vi "CP Selection for Plot and Graph_MS.vi"(7 "Sample cluster":T2, 8 "CP Profile Table":string[][](table), 9 "CP A Tag":string[](array[string]), 10 "Signal Tag AZ":string[](array[string]), 11 "Long Signal Profile Table A":string[][](table) caption="Long Singla Profile Table") -> (0 "CP A Tag AZ":string[](array[string]), 1 "Abs Plot Graph":dbl[][](graph), 2 "Plot Graph":dbl[][](graph), 3 "LCP Table":string[][](table), 5 "LAP":T1)   [LabVIEW 2018]
panel:
  out "LAP_Tag":string[](array[string])
  out "LAP Table":string[][](table) caption="LCP Table"
  out "M_Base Number":i32[](array[numeric])
  out "Direction":string[](array[string])
  out "Cutted Sequence":string
  out "Sample Sequence":string
  out "M_Seq EN":i32
  out "M_Seq SN":i32
  out "LS#":string[][](array[string])
  out "CP Profile Table for Bseq":string[][](table)
  out "CP Profile Table for All Seql":string[][](table)
  out "CP Profile Table for RSeq":string[][](table)
  out "読み取り開始番号":i32
  out "読み取り終了番号":i32
  out "Base Number":i32[](array[numeric])
  out "Seq EN":i32
  out "Seq SN":i32
  out "サイズ":i32
  out "Signal Profile Table":string[][](table) caption="Singla Profile Table"
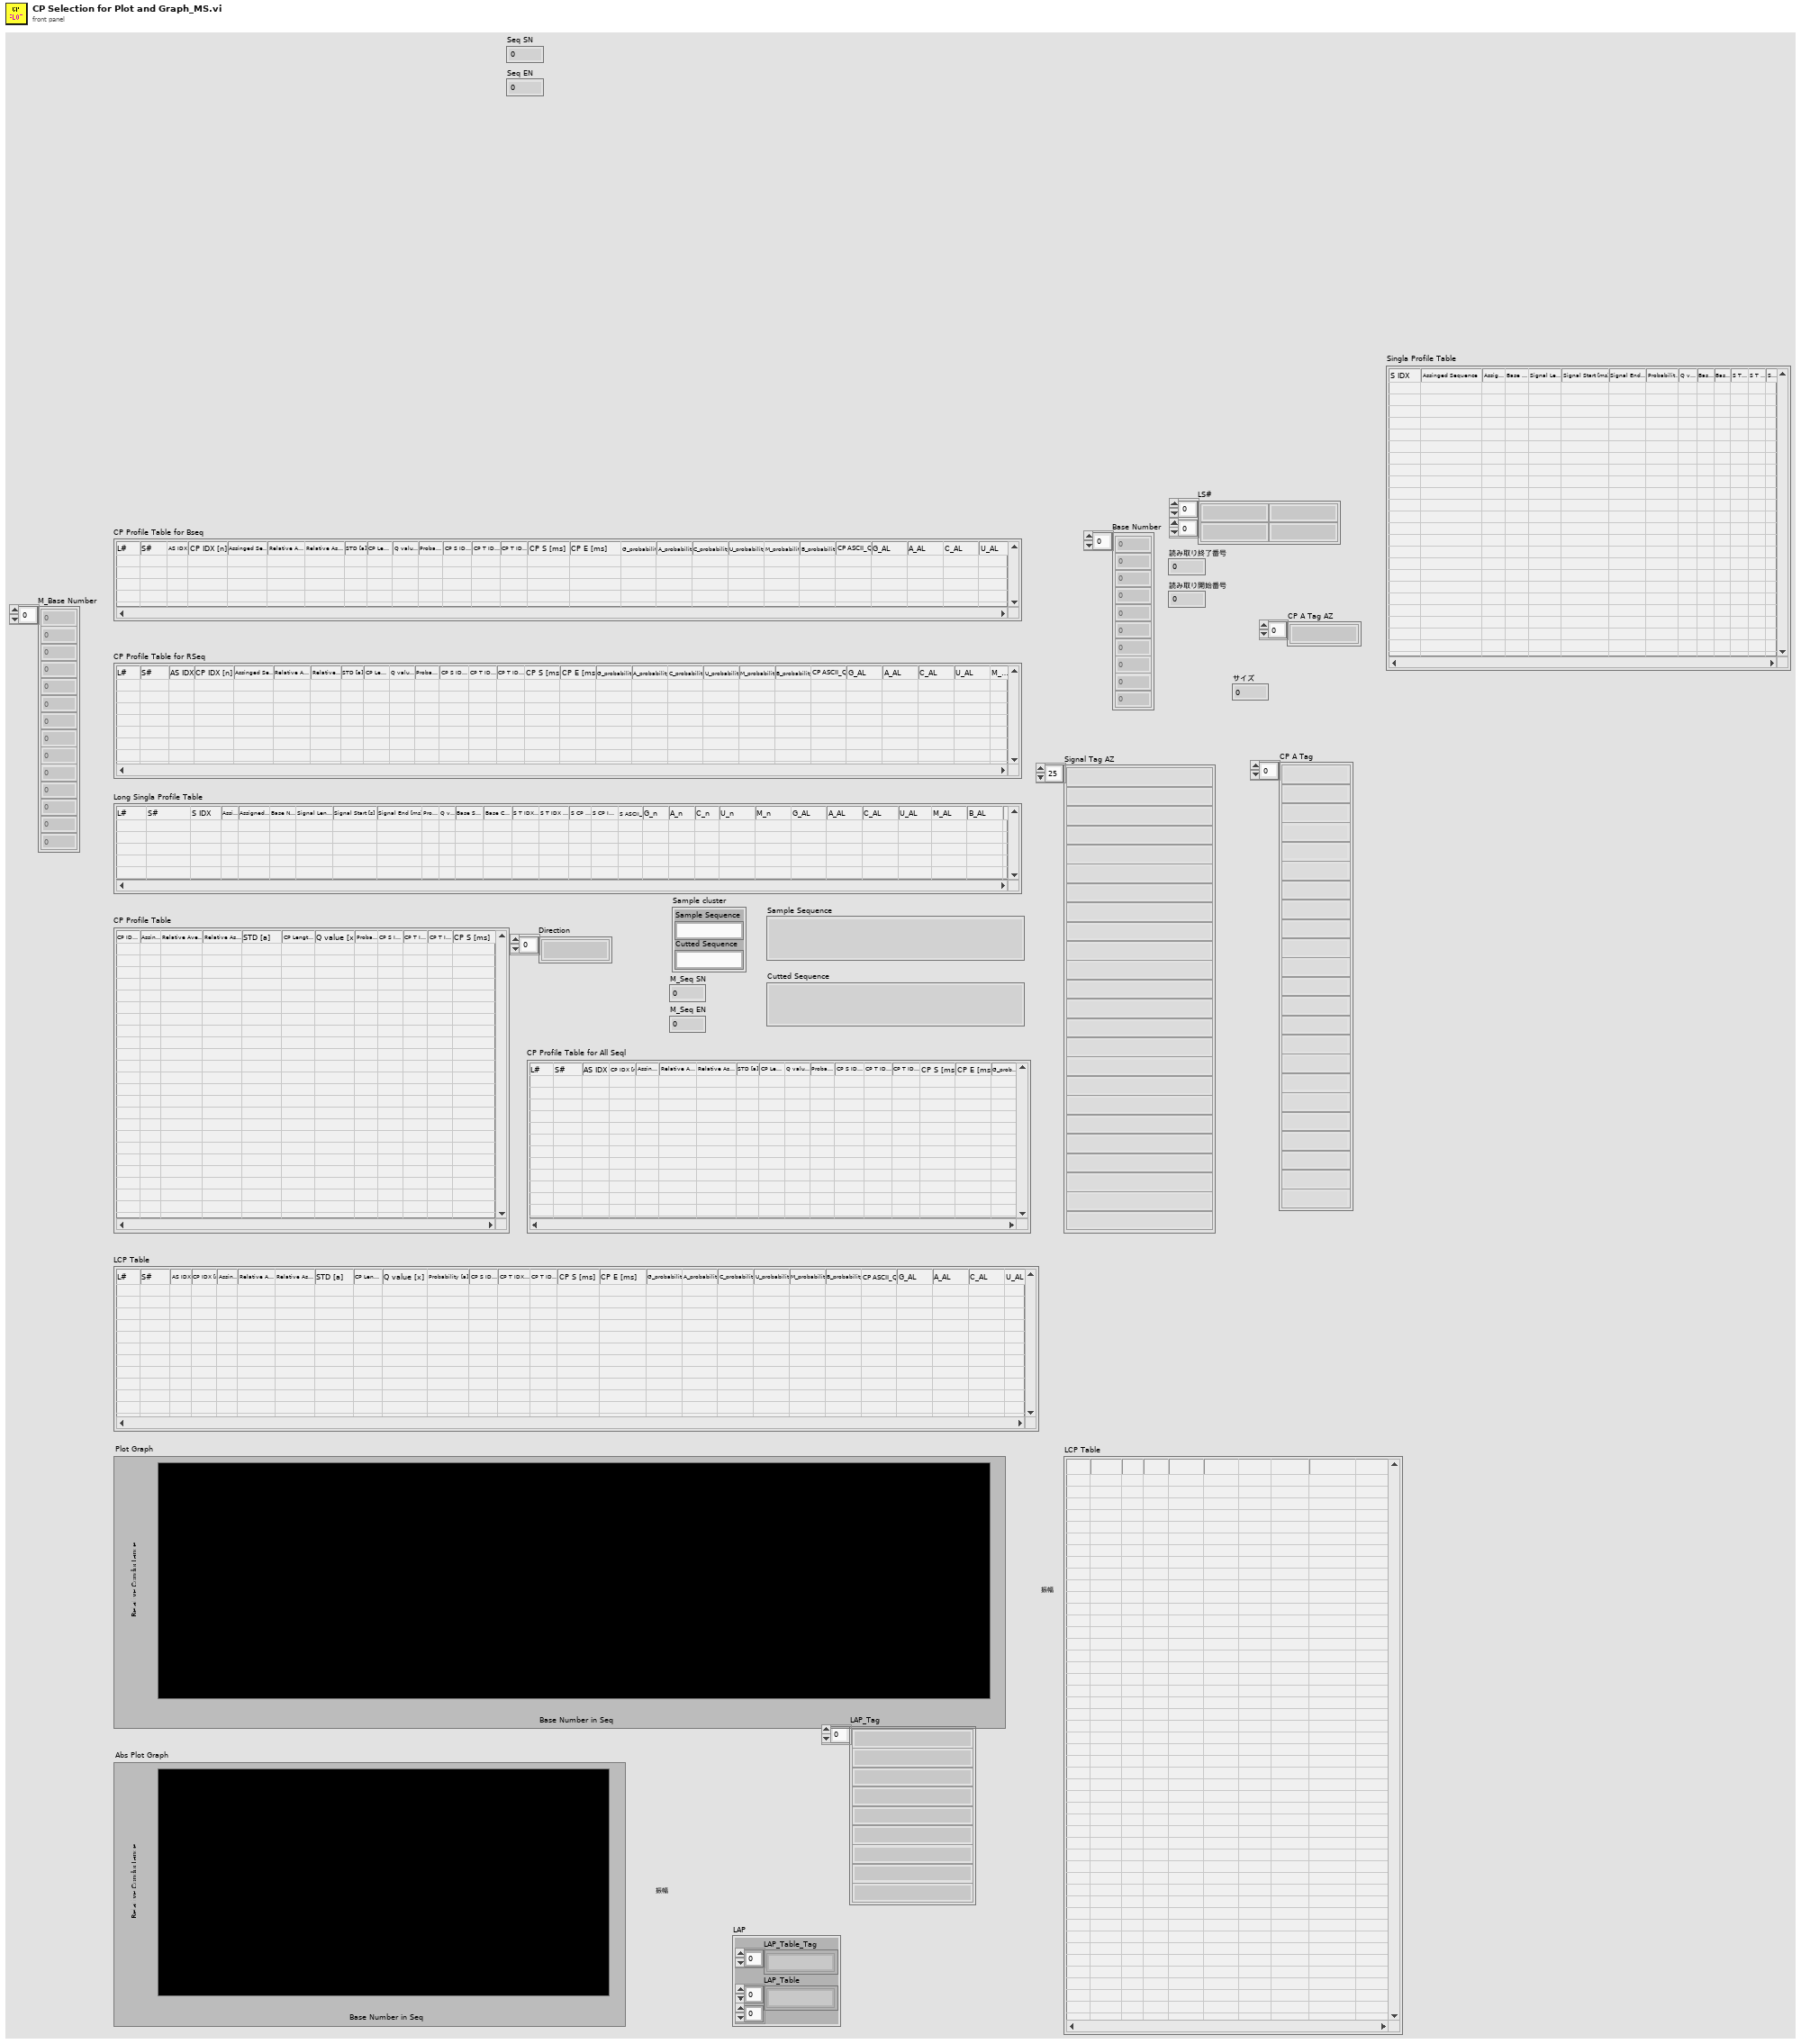
[diagram p1: front panel]
types:
  T1 = cluster{"LAP_Table_Tag":string[], "LAP_Table":string[][]}
  T2 = cluster{"Sample Sequence":string, "Cutted Sequence":string}
  T3 = cluster{"S CP IDX Start [n]":string[], "S CP IDX End [n]":string[], "Assinged Sequence":string[], "Direction":string[], "Mx Right Read Seq":string[], "Seq SNo":string[], "Seq ENo":string[], "Front Seq":string[], "Seq":string[], "Later Seq":string[], "MSeq_SNo":string[], "MSeq_ENo":string[], "L# [n]":string[], "S# [n]":string[], "M_RRead_Seq":string[], "M_MxRight_No":string[]}
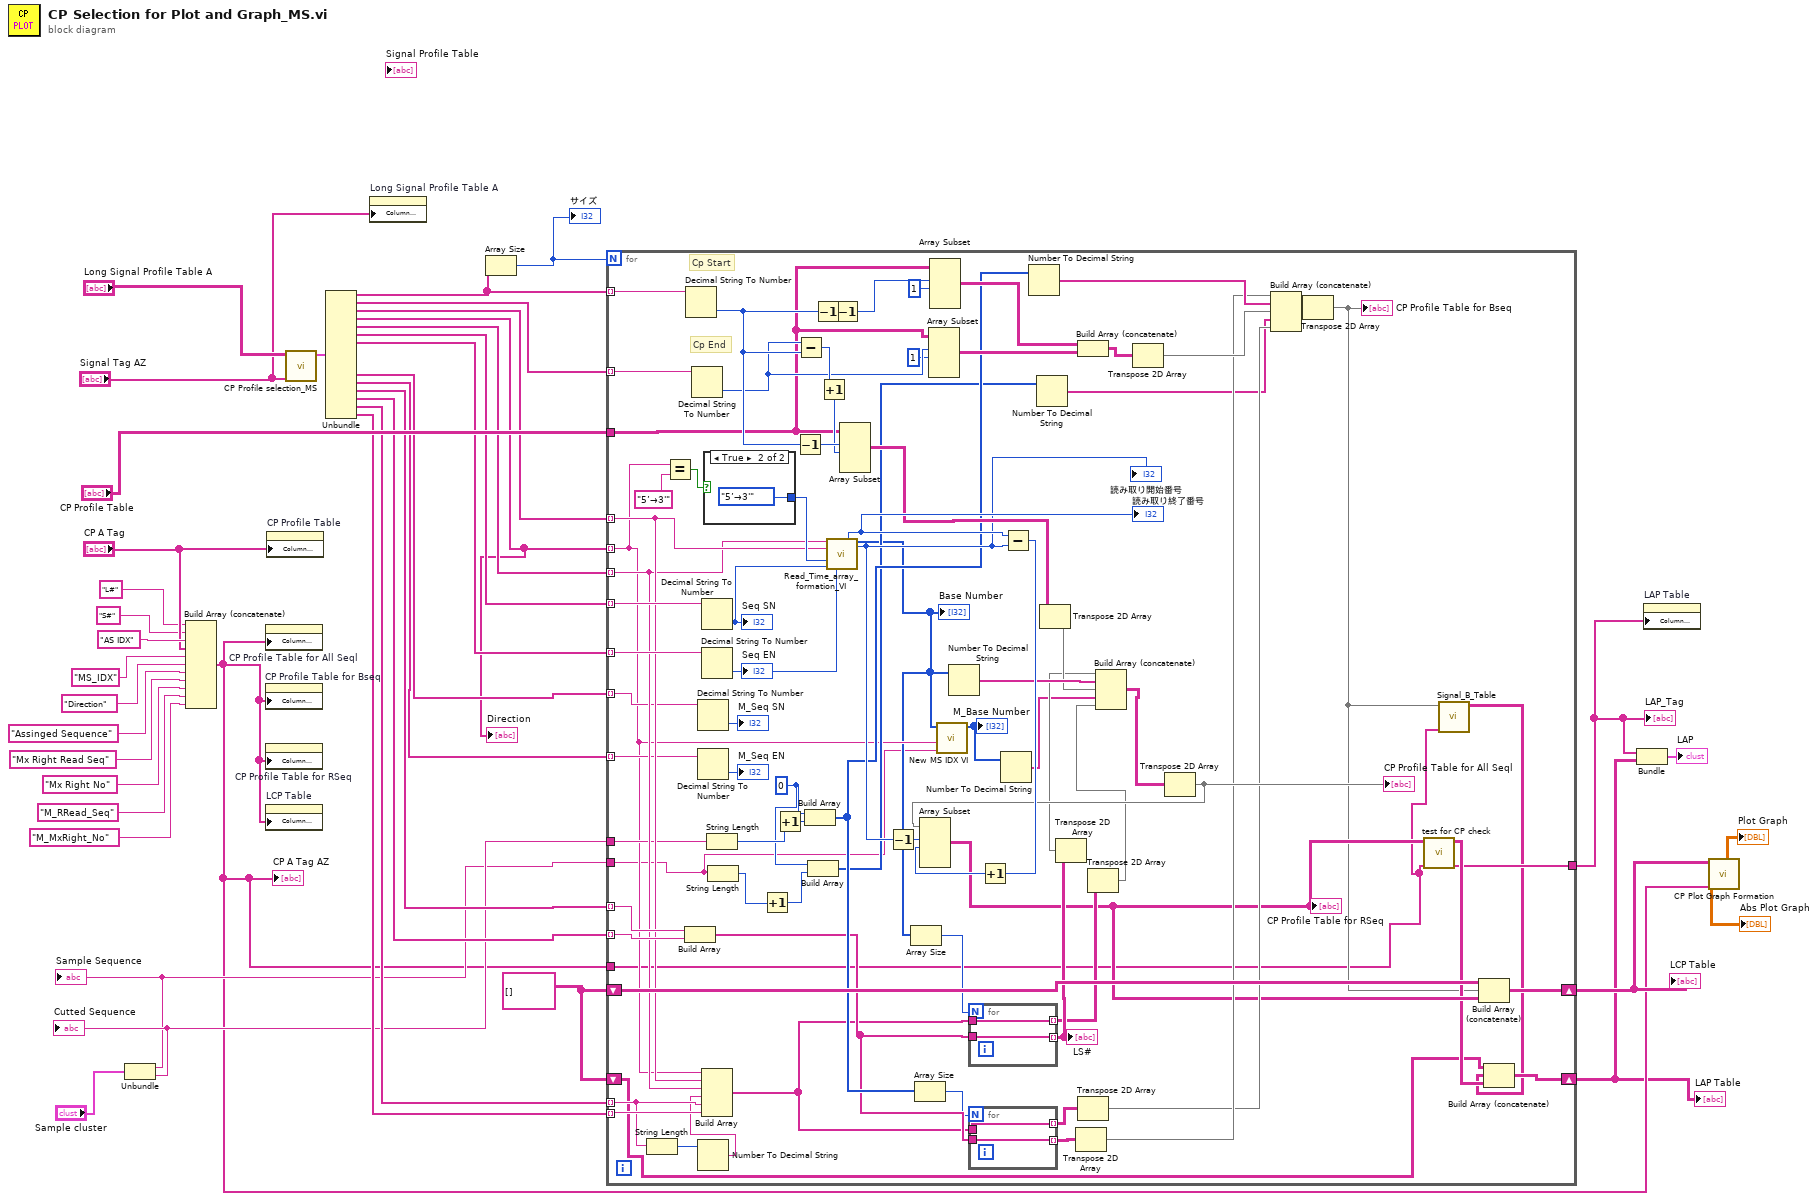
[diagram p0: block diagram]
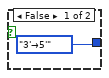
[diagram p2: hidden frame]
diagram:
  w4 = string[][] []
  n1 = Unbundle("Sample cluster") -> ("Sample Sequence"=w8:string, "Cutted Sequence"=w9:string)
  "Sample Sequence" <- w8
  "Cutted Sequence" <- w9
  n2 = Build Array (concatenate)("L#" ("y"), "S#" ("y"), "AS IDX" ("y"), "CP A Tag", "MS_IDX" ("y"), "Direction" ("y"), "Assinged Sequence" ("y"), "Mx Right Read Seq" ("y"), "Mx Right No" ("y"), "M_RRead_Seq" ("y"), "M_MxRight_No" ("y")) -> (w5:string[])
  "CP A Tag AZ" <- w5
  n3 = property on="CP Profile Table for All Seql" class="Tbl (strict)"("Column Headers[]"=w5) -> ()  [unwired: 2 in, 2 out]
  n4 = property on="CP Profile Table for Bseq" class="Tbl (strict)"("Column Headers[]"=w5) -> ()  [unwired: 2 in, 2 out]
  n5 = property on="CP Profile Table for RSeq" class="Tbl (strict)"("Column Headers[]"=w5) -> ()  [unwired: 2 in, 2 out]
  n6 = property on="LCP Table" class="Tbl (strict)"("Column Headers[]"=w5) -> ()  [unwired: 2 in, 2 out]
  n7 = property on="CP Profile Table" class="Tbl (strict)"("Column Headers[]"="CP A Tag") -> ()  [unwired: 2 in, 2 out]
  n8 = call "CP Profile selection_MS.vi"("Signal Tag AZ"="Signal Tag AZ", "Long Signal Profile Table A"="Long Signal Profile Table A") -> ("CP selected IDX"=w22:T3)  [unwired: 9 in]
  n9 = Unbundle(w22) -> ("S CP IDX Start [n]"=w36:string[], "S CP IDX End [n]"=w38:string[], "Assinged Sequence"=w37:string[], "Direction"=w7:string[], "Mx Right Read Seq"=w35:string[], "Seq SNo"=w34:string[], "Seq ENo"=w33:string[], "MSeq_SNo"=w12:string[], "MSeq_ENo"=w11:string[], "L# [n]"=w29:string[], "S# [n]"=w28:string[], "M_RRead_Seq"=w14:string[], "M_MxRight_No"=w13:string[])  [unwired: 3 out]
  "Direction" <- w7
  n10 = property on="Long Signal Profile Table A" class="Tbl (strict)"("Column Headers[]"="Signal Tag AZ") -> ()  [unwired: 2 in, 2 out]
  n11 = Array Size(array=w36) -> (size(s)=w40:i32)
  "サイズ" <- w40
  n12 = for {
    N: w40 -> [_]
    tunnel: w36 -> [w123] mode=indexing
    tunnel: w38 -> [w122] mode=indexing
    tunnel: "CP Profile Table" -> [w102]
    tunnel: w37 -> [w74] mode=indexing
    tunnel: w35 -> [w73] mode=indexing
    tunnel: w34 -> [w118] mode=indexing
    tunnel: w33 -> [w117] mode=indexing
    tunnel: w7 -> [w54] mode=indexing
    shift-right: [w85] -> w6
    shift-left: w4 -> [w86]
    tunnel: w29 -> [w84] mode=indexing
    tunnel: w28 -> [w83] mode=indexing
    tunnel: w14 -> [w68] mode=indexing
    tunnel: w13 -> [w69] mode=indexing
    tunnel: w12 -> [w63] mode=indexing
    tunnel: w11 -> [w62] mode=indexing
    tunnel: w9 -> [w61]
    tunnel: w8 -> [w52]
    tunnel: w5 -> [w43]
    shift-right: [w46] -> w2
    shift-left: w4 -> [w42]
    tunnel: [w45] -> w3
    w60 = 0
    # "Cp End"
    # "Cp Start"
    n13 = String Length(string=w68) -> (length=w67:i32)
    n14 = Equal?(x=w54, y="5’→3'") -> (x = y?=w112:bool)
    n15 = Build Array(w84, w83) -> (w78:string[])
    n16 = Decimal String To Number(string=w123) -> (number=w107:i32)  [unwired: 2 in, 1 out]
    n17 = Decimal String To Number(string=w122) -> (number=w103:i32)  [unwired: 2 in, 1 out]
    n18 = Decimal String To Number(string=w63) -> (number=→"M_Seq SN":i32)  [unwired: 2 in, 1 out]
    n19 = Decimal String To Number(string=w62) -> (number=→"M_Seq EN":i32)  [unwired: 2 in, 1 out]
    n20 = Number To Decimal String(number=w67) -> (decimal integer string=w66:string)  [unwired: 1 in]
    n21 = Decimal String To Number(string=w118) -> (number=w116:i32)  [unwired: 2 in, 1 out]
    "Seq SN" <- w116
    n22 = Decimal String To Number(string=w117) -> (number=w115:i32)  [unwired: 2 in, 1 out]
    "Seq EN" <- w115
    n23 = Build Array(w54, w74, w73, w66, w68, w69) -> (w72:string[])
    n24 = case shown="True" w112 {
      tunnel: [enum16{"5’→3'", "3'→5'"}."3'→5'" ("リード方向総合") enum16{"5’→3'", "3'→5'"}."5’→3'" ("リード方向総合")] -> w114
      frame False {
      }
      frame True {
      }
    }
    n25 = String Length(string=w61) -> (length=w95:i32)
    n26 = String Length(string=w52) -> (length=w59:i32)
    n27 = Increment(x=w59) -> (x+1=w58:i32)
    n28 = Increment(x=w95) -> (x+1=w88:i32)
    n29 = Decrement(x=w107) -> (x-1=w121:i32)
    n30 = Subtract(x=w103, y=w107) -> (x-y=w120:i32)
    n31 = Build Array(w60, w88) -> (w79:i32[])
    n32 = Build Array(w60, w58) -> (w57:i32[])
    n33 = Decrement(x=w107) -> (x-1=w105:i32)
    n34 = Increment(x=w120) -> (x+1=w119:i32)
    n35 = call "Read_Time_array_formation_VI.vi"("Right Read MAX"=w73, "読み取り配列"=w74, "リード方向総合"=w114, "配列開始番号"=w116, "配列終了番号"=w115) -> ("読み取り開始番号"=w96:i32, "読み取り終了番号"=w110:i32, "Base Number"=w53:i32[])  [unwired: 3 in, 5 out]
    "Base Number" <- w53
    "読み取り終了番号" <- w110
    "読み取り開始番号" <- w96
    n36 = Decrement(x=w105) -> (x-1=w104:i32)
    n37 = Array Subset(array=w102, index (row)=w121, length (row)=w119) -> (w99:string[][])  [unwired: 2 in]
    n38 = Decrement(x=w96) -> (x-1=w111:i32)
    n39 = Array Size(array=w53) -> (size(s)=w82:i32)
    n40 = Array Size(array=w79) -> (size(s)=w77:i32)
    n41 = Array Subset(array=w102, index (row)=w103, length (row)=1 ("長さ")) -> (w93:string[][])  [unwired: 2 in]
    n42 = Array Subset(array=w102, index (row)=w104, length (row)=1 ("長さ")) -> (w94:string[][])  [unwired: 2 in]
    n43 = call "New MS IDX VI.vi"("Sample Sequence"=w52, "Direction"=w54, "Base Number"=w53) -> ("Array"=w51:i32[])  [unwired: 8 in]
    "M_Base Number" <- w51
    n44 = Number To Decimal String(number=w53) -> (decimal integer string=w98:string[])  [unwired: 1 in]
    n45 = for {
      N: w82 -> [_]
      tunnel: w78 -> [w127]
      tunnel: [w127] -> w81 mode=indexing
      tunnel: w72 -> [w126]
      tunnel: [w126] -> w71 mode=indexing
    }
    "LS#" <- w81
    n46 = for {
      N: w77 -> [_]
      tunnel: w78 -> [w125]
      tunnel: [w125] -> w76 mode=indexing
      tunnel: [w124] -> w70 mode=indexing
      tunnel: w72 -> [w124]
    }
    n47 = Number To Decimal String(number=w51) -> (decimal integer string=w49:string[])  [unwired: 1 in]
    n48 = Subtract(x=w110, y=w96) -> (x-y=w109:i32)
    n49 = Increment(x=w109) -> (x+1=w108:i32)
    n50 = Number To Decimal String(number=w79) -> (decimal integer string=w91:string[])  [unwired: 1 in]
    n51 = Number To Decimal String(number=w57) -> (decimal integer string=w55:string[])  [unwired: 1 in]
    n52 = Transpose 2D Array(2D array=w99) -> (transposed array=w97:string[][])
    n53 = Transpose 2D Array(2D array=w81) -> (transposed array=w80:string[][])
    n54 = Transpose 2D Array(2D array=w76) -> (transposed array=w75:string[][])
    n55 = Build Array (concatenate)(w94, w93) -> (w92:string[][])
    n56 = Transpose 2D Array(2D array=w70) -> (transposed array=w56:string[][])
    n57 = Transpose 2D Array(2D array=w71) -> (transposed array=w50:string[][])
    n58 = Build Array (concatenate)(w80, w98, w97, w49, w50) -> (w100:string[][])
    n59 = Transpose 2D Array(2D array=w92) -> (transposed array=w90:string[][])
    n60 = Transpose 2D Array(2D array=w100) -> (transposed array=w87:string[][])
    "CP Profile Table for All Seql" <- w87
    n61 = Array Subset(array=w87, index (row)=w111, length (row)=w108) -> (w48:string[][])  [unwired: 2 in]
    "CP Profile Table for RSeq" <- w48
    n62 = Build Array (concatenate)(w75, w91, w90, w55, w56) -> (w89:string[][])
    n63 = Transpose 2D Array(2D array=w89) -> (transposed array=w44:string[][])
    "CP Profile Table for Bseq" <- w44
    n64 = call "test for CP check.vi"("CP A Tag AZ"=w43, "CP Profile Table for RSeq"=w48) -> ("LAP_Tag"=w45:string[], "Base Table RSeq"=w47:string[][])  [unwired: 8 in]
    n65 = call "Signal_B_Table.vi"("CP A Tag AZ"=w43, "CP Profile Table for Bseq"=w44) -> ("ACP Table"=w41:string[][])  [unwired: 9 in]
    n66 = Build Array (concatenate)(w86, w44, w48) -> (w85:string[][])
    n67 = Build Array (concatenate)(w42, w41, w47) -> (w46:string[][])
  }
  "LCP Table" <- w6
  "LAP Table" <- w2
  "LAP_Tag" <- w3
  n68 = Bundle("LAP_Tag"=w3, w2) -> (→"LAP":cluster{"LAP_Tag":string[], string[][]})  [unwired: 1 in]
  n69 = property on="LAP Table" class="Tbl (strict)"("Column Headers[]"=w3) -> ()  [unwired: 2 in, 2 out]
  n70 = call "CP Plot Graph Formation.vi"("CP A Tag AZ"=w5, "CP Profile Table for plot"=w6) -> ("Plot Graph"=→"Plot Graph":dbl[][], "Abs Plot Graph"=→"Abs Plot Graph":dbl[][])  [unwired: 2 in, 6 out]
